vi "RemoteVI Window Popup Info.vi"(0 "hWnd":u64, 11 "error in":errorcluster) -> (4 "popup?":bool, 6 "window":T1, 15 "error out":errorcluster)   [LabVIEW 2020, in "RemoteVI.lvlib"]
doc: "Reads the class, style and screen rectangle of the top-level window hWnd and decides whether it looks like a LabVIEW popup that FP.Get Image cannot see: visible AND (class LVMenuWnd OR (style has WS_POPUP 0x80000000 AND no WS_CAPTION 0x00C00000 AND a non-empty rectangle)). Win32 calls only (IsWindowVisible, GetClassNameW, GetWindowLongPtrW GWL_STYLE, GetWindowRect), no VI Server, so it works while LabVIEW's UI thread is blocked. Used by RemoteVI Find Popups.vi for each of LabVIEW's own windows."
uses:
  RemoteVI.lvlib
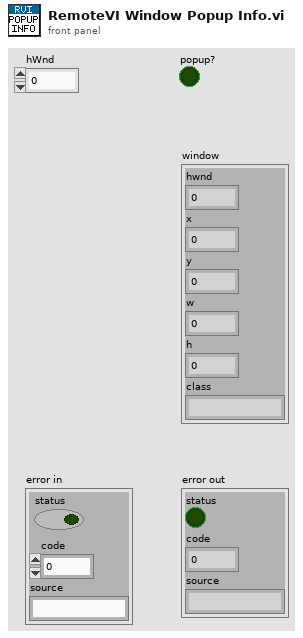
[diagram p1: front panel]
types:
  T1 = cluster{"hwnd":u64, "x":i32, "y":i32, "w":i32, "h":i32, "class":string}
  T2 = cluster{"left":i32, "top":i32, "right":i32, "bottom":i32}
  T3 = cluster{"hWnd":u64, "left":i32, "top":i32, i32, i32, "class name":string}
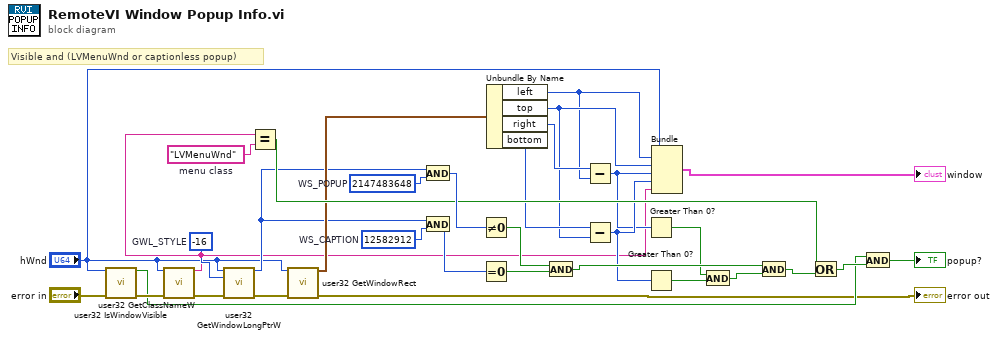
[diagram p0: block diagram]
diagram:
  w23 = i64 12582912  # WS_CAPTION
  w22 = i64 2147483648  # WS_POPUP
  w20 = "LVMenuWnd"  # menu class
  w10 = -16  # GWL_STYLE
  # "Visible and (LVMenuWnd or captionless popup)"
  n1 = call "user32 IsWindowVisible.vi"("hWnd"="hWnd", "error in"="error in") -> ("visible?"=w6:bool, "error out"=w7:errorcluster)  [unwired: 12 in]
  n2 = call "user32 GetClassNameW.vi"("hWnd"="hWnd", "error in"=w7) -> ("class name"=w8:string, "error out"=w9:errorcluster)  [unwired: 11 in, 1 out]
  n3 = call "user32 GetWindowLongPtrW.vi"("hWnd"="hWnd", "nIndex"=w10, "error in"=w9) -> ("return value"=w11:i64, "error out"=w12:errorcluster)  [unwired: 11 in]
  n4 = Equal?(x=w8, y=w20) -> (x = y?=w21:bool)
  n5 = call "user32 GetWindowRect.vi"("hWnd"="hWnd", "error in"=w12) -> ("RECT"=w13:T2, "error out"=→"error out":errorcluster)  [unwired: 11 in, 1 out]
  n6 = And(x=w11, y=w22) -> (x .and. y?=w24:i64)
  n7 = And(x=w11, y=w23) -> (x .and. y?=w25:i64)
  n8 = Not Equal To 0?(x=w24) -> (x != 0?=w26:bool)
  n9 = Equal To 0?(x=w25) -> (x = 0?=w27:bool)
  n10 = Unbundle By Name(w13) -> ("left"=w14:i32, "top"=w15:i32, "right"=w16:i32, "bottom"=w17:i32)
  n11 = And(x=w26, y=w27) -> (x .and. y?=w30:bool)
  n12 = Subtract(x=w16, y=w14) -> (x-y=w18:i32)
  n13 = Subtract(x=w17, y=w15) -> (x-y=w19:i32)
  n14 = Greater Than 0?(x=w18) -> (x > 0?=w28:bool)
  n15 = Greater Than 0?(x=w19) -> (x > 0?=w29:bool)
  n16 = Bundle("hWnd"="hWnd", "left"=w14, "top"=w15, w18, w19, "class name"=w8) -> (→"window":T3)  [unwired: 1 in]
  n17 = And(x=w28, y=w29) -> (x .and. y?=w31:bool)
  n18 = And(x=w30, y=w31) -> (x .and. y?=w32:bool)
  n19 = Or(x=w21, y=w32) -> (x .or. y?=w33:bool)
  n20 = And(x=w6, y=w33) -> (x .and. y?=→"popup?":bool)
